vi "Read Object String Property.vi"(8 "error in":errorcluster, 10 "property name":string, 11 "object in":T1) -> (0 "error out":errorcluster, 2 "text":string, 3 "object out":T1)   [LabVIEW 2026, in "ToastNotification.lvlib" / "Reflection DotNet.lvlib"]
doc: "Read a named property from a borrowed .NET object, copy its ToString representation and release the acquired boxed property value on success and failure. object out is the original borrowed alias, preserved on incoming error. Does not close the input object. A null property value produces a conversion error rather than an implicit empty-string substitution."
uses:
  Reflection DotNet.lvlib
  Callback Object Reference.ctl
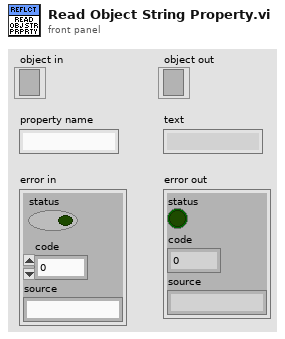
[diagram p1: front panel]
types:
  T1 = typedef "ToastNotification.lvlib/Reflection DotNet.lvlib/Callback Object Reference.ctl" = refnum<k24>
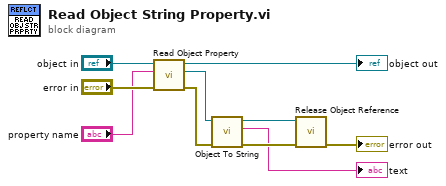
[diagram p0: block diagram]
diagram:
  n1 = call "Read Object Property.vi"("error in"="error in", "property name"="property name", "object in"="object in") -> ("error out"=w3:errorcluster, "value"=w2:T1, "object out"=→"object out":T1)  [unwired: 6 in]
  n2 = call "Object To String.vi"("error in (no error)"=w3, "Object in"=w2) -> ("error out"=w9:errorcluster, "Text"=→"text":string, "Object out"=w1:refnum<k24>)  [unwired: 7 in]
  n3 = call "Release Object Reference.vi"("error in"=w9, "object"=w1) -> ("error out"=→"error out":errorcluster)  [unwired: 9 in]
